vi "List Roots.vi"(10 "Optional Root Name":string, 11 "Tree Map In":T1) -> (3 "Unique Root Paths Set":set{string}(c389))   [LabVIEW 2019, in "Tree Map.lvlib"]
doc: "Iterates through all tree nodes and finds the root nodes. This feature is designed only for the Tree Map, since an XML document cannot contain more than 1 root.\n\n<b>Author:</b> Piotr Kruczkowski <PrimaryKey>\n<b>License:</b> NewBSD\n\nCopyright (c) 2019, National Instruments\nAll rights reserved.\n\nRedistribution and use in source and binary forms, with or without\nmodification, are permitted provided that the following conditions are met:\n1. Redistributions of source code must retain the above copyright\n notice, this list of conditions and the following disclaimer.\n2. Redistributions in binary form must reproduce the above copyright\n notice, this list of conditions and the following disclaimer in the\n documentation and/or other materials provided with the distribution.\n3. Neither the name of National Instruments nor the\n names of its contributors may be used to endorse or promote products\n derived from this software without specific prior written permission.\n\nTHIS SOFTWARE IS PROVIDED BY National Instruments ''AS IS'' AND ANY\nEXPRESS OR IMPLIED WARRANTIES, INCLUDING, BUT NOT LIMITED TO, THE IMPLIED\nWARRANTIES OF MERCHANTABILITY AND FITNESS FOR A PARTICULAR PURPOSE ARE\nDISCLAIMED. IN NO EVENT SHALL National Instruments BE LIABLE FOR ANY\nDIRECT, INDIRECT, INCIDENTAL, SPECIAL, EXEMPLARY, OR CONSEQUENTIAL DAMAGES\n(INCLUDING, BUT NOT LIMITED TO, PROCUREMENT OF SUBSTITUTE GOODS OR SERVICES;\nLOSS OF USE, DATA, OR PROFITS; OR BUSINESS INTERRUPTION) HOWEVER CAUSED AND\nON ANY THEORY OF LIABILITY, WHETHER IN CONTRACT, STRICT LIABILITY, OR TORT\n(INCLUDING NEGLIGENCE OR OTHERWISE) ARISING IN ANY WAY OUT OF THE USE OF THIS\nSOFTWARE, EVEN IF ADVISED OF THE POSSIBILITY OF SUCH DAMAGE."
uses:
  Tree Map.lvlib
  Tree Map Data.ctl
  Utility/Join Strings Tree.vi
  SubVIs/TM Head and Tail.vi
  SubVIs/TM Init and Last.vi
  Utility/Split String Tree.vi
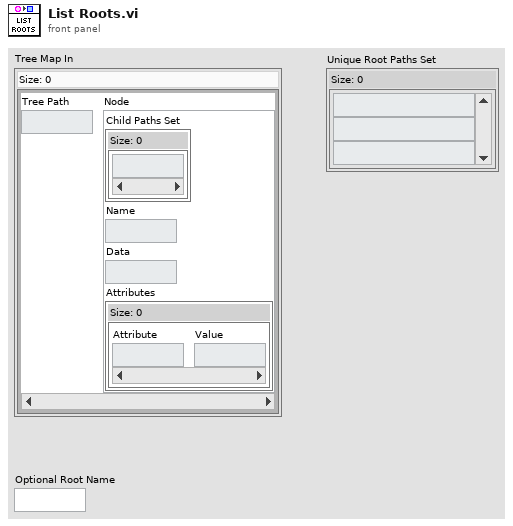
[diagram p1: front panel]
types:
  T1 = typedef "Tree Map.lvlib/Tree Map Data.ctl" = map{string, cluster{"Child Paths Set":set{string}, "Name":string, "Data":string, "Attributes":map{string, string}}}
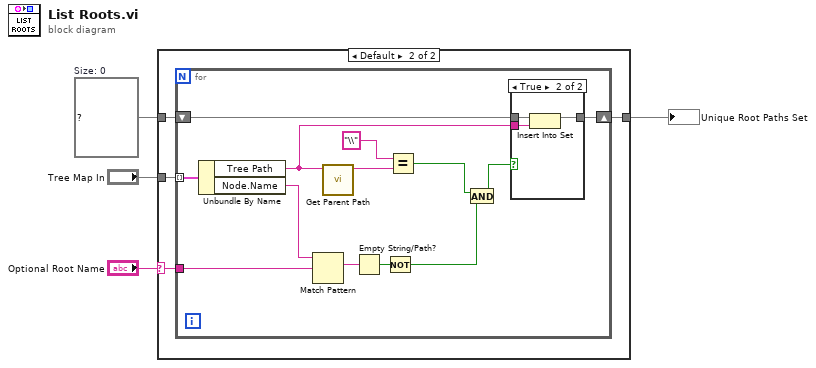
[diagram p0: block diagram]
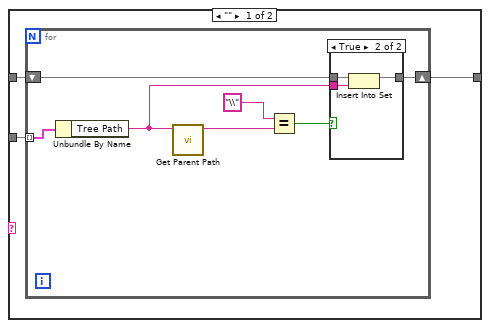
[diagram p2: hidden frame]
diagram:
  w3 = set{string} {}  # Size: 0
  n1 = case shown="Default" "Optional Root Name" {
    selector: "Optional Root Name" -> [_ w19]
    tunnel: "Tree Map In" -> [w5 w22]
    tunnel: w3 -> [w7 w21]
    tunnel: [w6 w20] -> w2
    frame "" {
      n2 = for {
        tunnel: w5 -> [w14] mode=indexing
        shift-right: [w12] -> w6
        shift-left: w7 -> [w11]
        n3 = Unbundle By Name(w14) -> ("Tree Path"=w13:string)
        n4 = call "Get Parent Path.vi"("Node Path"=w13) -> ("Parent Path"=w9:string)  [unwired: 8 in, 2 out]
        n5 = Equal?(x="\\", y=w9) -> (x = y?=w8:bool)
        n6 = case shown="True" w8 {
          tunnel: w13 -> [_ w18]
          tunnel: [w15 w17] -> w12
          tunnel: w11 -> [w15 w16]
          frame False {
          }
          frame True {
            n7 = Insert Into Set(10:w18, 11:w16) -> (3:w17:set{string})  [unwired: 1 out]
          }
        }
      }
    }
    frame Default {
      n8 = for {
        tunnel: w22 -> [w35] mode=indexing
        shift-right: [w33] -> w20
        shift-left: w21 -> [w32]
        tunnel: w19 -> [w30]
        n9 = Unbundle By Name(w35) -> ("Tree Path"=w34:string, "Node.Name"=w29:string)
        n10 = Match Pattern(string=w29, regular expression=w30) -> (match substring=w31:string)  [unwired: 1 in, 3 out]
        n11 = call "Get Parent Path.vi"("Node Path"=w34) -> ("Parent Path"=w25:string)  [unwired: 8 in, 2 out]
        n12 = Empty String/Path?(string/path=w31) -> (empty?=w28:bool)
        n13 = Not(x=w28) -> (.not. x?=w26:bool)
        n14 = Equal?(x="\\", y=w25) -> (x = y?=w23:bool)
        n15 = And(x=w23, y=w26) -> (x .and. y?=w27:bool)
        n16 = case shown="True" w27 {
          tunnel: w34 -> [_ w39]
          tunnel: [w36 w38] -> w33
          tunnel: w32 -> [w36 w37]
          frame False {
          }
          frame True {
            n17 = Insert Into Set(10:w39, 11:w37) -> (3:w38:set{string})  [unwired: 1 out]
          }
        }
      }
    }
  }
  "Unique Root Paths Set" <- w2
